vi "RemoteVI Track Modifiers.vi"(0 "kind":T1(ring), 5 "msg":u32, 7 "wParam":u64, 9 "mods in":u8) -> (4 "mods out":u8)   [LabVIEW 2020, in "RemoteVI.lvlib"]
doc: "Keeps the modifier keys the remote user holds, per client (docs\\protocol.md section 4.4). mods is a bit set: 1 Shift, 2 Ctrl, 4 Alt. A key message WM_KEYDOWN (256) of VK_SHIFT 0x10, VK_LSHIFT 0xA0 or VK_RSHIFT 0xA1 sets bit 1 and its WM_KEYUP (257) clears it - likewise 0x11/0xA2/0xA3 for Ctrl (bit 2) and 0x12/0xA4/0xA5 for Alt (bit 4). An allowed mouse message (512-522) carries the whole Shift and Ctrl state in wParam: bit 1 = MK_SHIFT (4), bit 2 = MK_CONTROL (8); Alt is kept. Anything else leaves mods unchanged. The server writes the result into the key state of LabVIEW's UI thread (RemoteVI Set Modifier Keys.vi) before posting, because LabVIEW reads the modifiers with GetKeyState and posted messages do not change that state (measured). Pure; reference trackModifiers() in tools\\lib\\input.mjs, vectors tests\\vectors\\translate.json (modifiers)."
uses:
  RemoteVI.lvlib
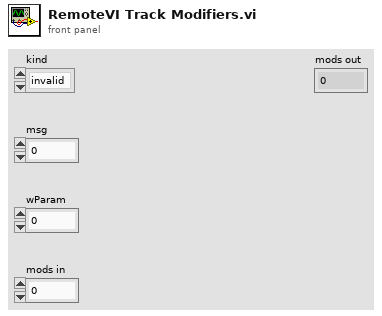
[diagram p1: front panel]
types:
  T1 = enum16{"invalid", "mouse", "key", "ack", "close", "splitter"}
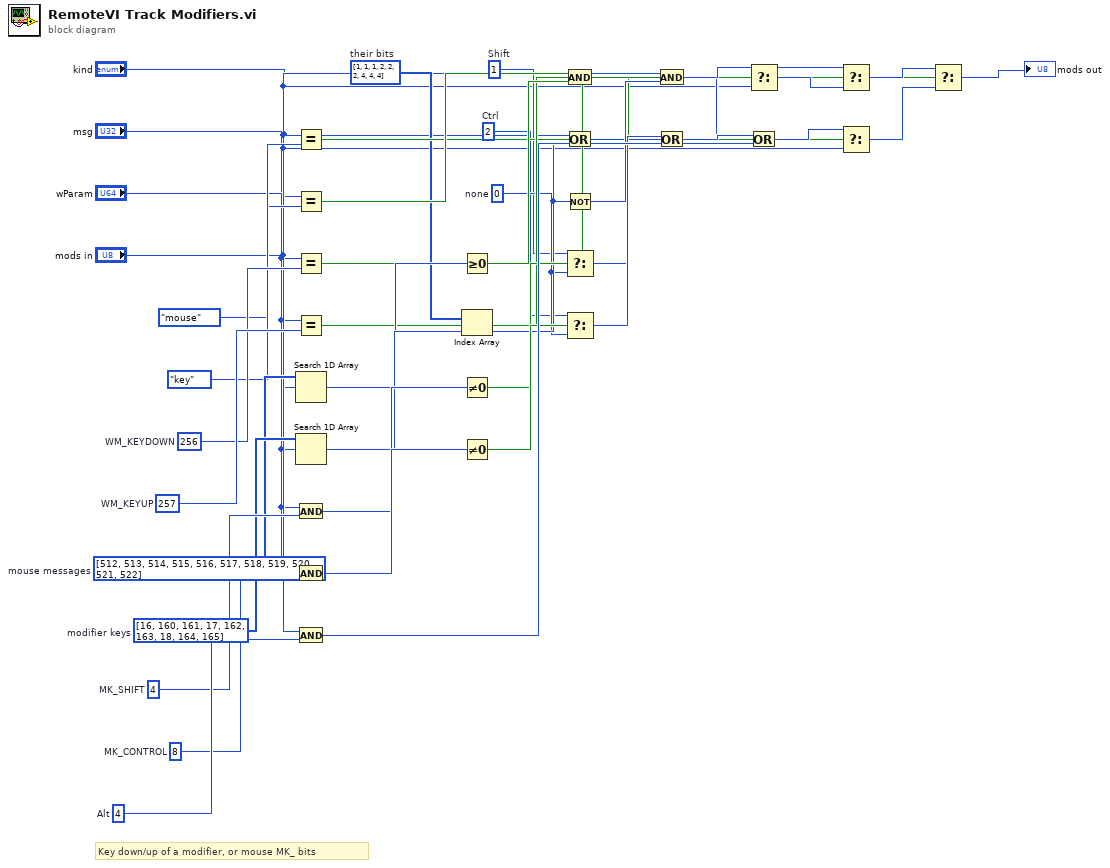
[diagram p0: block diagram]
diagram:
  w18 = u8 0  # none
  w17 = u8 4  # Alt
  w16 = u8 2  # Ctrl
  w15 = u8 1  # Shift
  w14 = u64 8  # MK_CONTROL
  w13 = u64 4  # MK_SHIFT
  w12 = u8[] [1, 1, 1, 2, 2, 2, 4, 4, 4]  # their bits
  w11 = u64[] [16, 160, 161, 17, 162, 163, 18, 164, 165]  # modifier keys
  w10 = u32[] [512, 513, 514, 515, 516, 517, 518, 519, 520, 521, 522]  # mouse messages
  w9 = u32 257  # WM_KEYUP
  w8 = u32 256  # WM_KEYDOWN
  # "Key down/up of a modifier, or mouse MK_ bits"
  n1 = Equal?(x="kind", y=T1."key") -> (x = y?=w19:bool)
  n2 = Equal?(x="kind", y=T1."mouse") -> (x = y?=w20:bool)
  n3 = Equal?(x="msg", y=w8) -> (x = y?=w21:bool)
  n4 = Equal?(x="msg", y=w9) -> (x = y?=w22:bool)
  n5 = Search 1D Array(1D array=w10, element="msg") -> (index of element=w23:i32)  [unwired: 1 in]
  n6 = Search 1D Array(1D array=w11, element="wParam") -> (index of element=w26:i32)  [unwired: 1 in]
  n7 = And(x="wParam", y=w13) -> (x .and. y?=w33:u64)
  n8 = And(x="wParam", y=w14) -> (x .and. y?=w34:u64)
  n9 = And(x="mods in", y=w17) -> (x .and. y?=w39:u8)
  n10 = Greater Or Equal To 0?(x=w23) -> (x >= 0?=w24:bool)
  n11 = Index Array(array=w12, index=w26) -> (element=w27:u8)
  n12 = Not Equal To 0?(x=w33) -> (x != 0?=w35:bool)
  n13 = Not Equal To 0?(x=w34) -> (x != 0?=w36:bool)
  n14 = And(x=w20, y=w24) -> (x .and. y?=w25:bool)
  n15 = Or(x="mods in", y=w27) -> (x .or. y?=w28:u8)
  n16 = Not(x=w27) -> (.not. x?=w29:u8)
  n17 = Select(t=w15, s=w35, f=w18) -> (s? t:f=w37:u8)
  n18 = Select(t=w16, s=w36, f=w18) -> (s? t:f=w38:u8)
  n19 = And(x="mods in", y=w29) -> (x .and. y?=w30:u8)
  n20 = Or(x=w37, y=w38) -> (x .or. y?=w40:u8)
  n21 = Select(t=w30, s=w22, f="mods in") -> (s? t:f=w31:u8)
  n22 = Or(x=w40, y=w39) -> (x .or. y?=w41:u8)
  n23 = Select(t=w28, s=w21, f=w31) -> (s? t:f=w32:u8)
  n24 = Select(t=w41, s=w25, f="mods in") -> (s? t:f=w42:u8)
  n25 = Select(t=w32, s=w19, f=w42) -> (s? t:f=→"mods out":u8)
